vi "From JSON.vi"(8 "error in (no error)":errorcluster, 10 "JSON":string, 11 "Double Float in":refnum<class "Abs_Time.lvclass">) -> (0 "error out":errorcluster, 3 "Double Float out":refnum<class "Abs_Time.lvclass">)   [LabVIEW 2021, in "Abs_Time.lvclass"]
uses:
  Abs_Time.lvclass
  Support/Type.ctl
  <vilib>/JDP Science/JSONtext/JSON text to Variant.vi
  <vilib>/JDP Science/JSONtext/LVClass Serializer/JSONtext LVClass Serializer.lvclass
  Abs_Time.lvclass/Abs_Time.ctl
  d9e1fb5e-ecfb-42bf-a4f8-ee95d664b313.vi
  Type/Abs_Type.lvclass
  Numeric/Abs_Numeric.lvclass
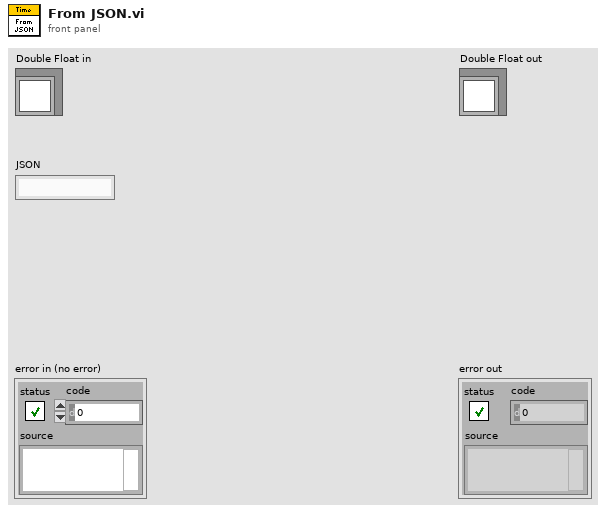
[diagram p1: front panel]
types:
  T1 = typedef "Abs_Time.lvclass/Type.ctl" = timestamp
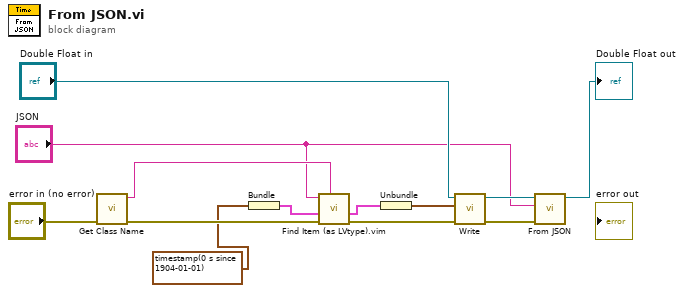
[diagram p0: block diagram]
diagram:
  n1 = call "Get Class Name.vi"("error in (no error)"="error in (no error)") -> ("error out"=w9:errorcluster, "class name"=w10:string)  [unwired: 9 in]
  n2 = Bundle(T1 timestamp(0 s since 1904-01-01)) -> (w11:cluster{T1})  [unwired: 1 in]
  n3 = call "Find Item (as LVtype).vim"("$Path or Item Name"=w10, "error in (no error)"=w9, "Data Type and Default Value"=w11, "JSON"="JSON") -> ("error out"=w5:errorcluster, "Data"=w12:cluster{T1})  [unwired: 4 in, 2 out]
  n4 = Unbundle(w12) -> (w6:T1)
  n5 = call-dynamic "Write.vi"("error in (no error)"=w5, "Value"=w6, "Double Float.lvclass_340760 in"="Double Float in") -> ("error out"=w4:errorcluster, "Double Float.lvclass_340760 out"=w3:refnum<class "Abs_Time.lvclass">)  [unwired: 7 in]
  n6 = call-parent "From JSON.vi"("error in (no error)"=w4, "JSON"="JSON", "Type in"=w3) -> ("Type out"=→"Double Float out":refnum<class "Abs_Time.lvclass">)  [unwired: 7 in, 1 out]
